vi "Global Log To String(Periodic Check).vi"(0 "Cross CSM Data":T3, 1 "Reset?":bool, 2 "Remove Immediately? (F)":bool, 3 "Time Format String":string="%<%H:%M:%S%3u>T", 9 "Settings":T2={"threashold(#/s)"=1.9, "Check Peroid(s)"=1.0}, 12 "Level (Normal)":T1) -> (4 "String":string, 10 "Periodic Info":string[](array[string]))   [LabVIEW 2017, in "Communicable State Machine.lvlib"]
uses:
  Communicable State Machine.lvlib
  _Support/Typedef/_CSM_GlobalLog_MSG.ctl
  _Support/Typedef/_CSM_Response Source Message.ctl
  _Support/Typedef/_CSM_GlobalLog_MSG_TYPE.ctl
  Periodic String Filter Setting.ctl
  _support/Periodic String Filter Level.ctl
  Periodic String Filter State.ctl
  _Shared/CSM Shared.lvlib
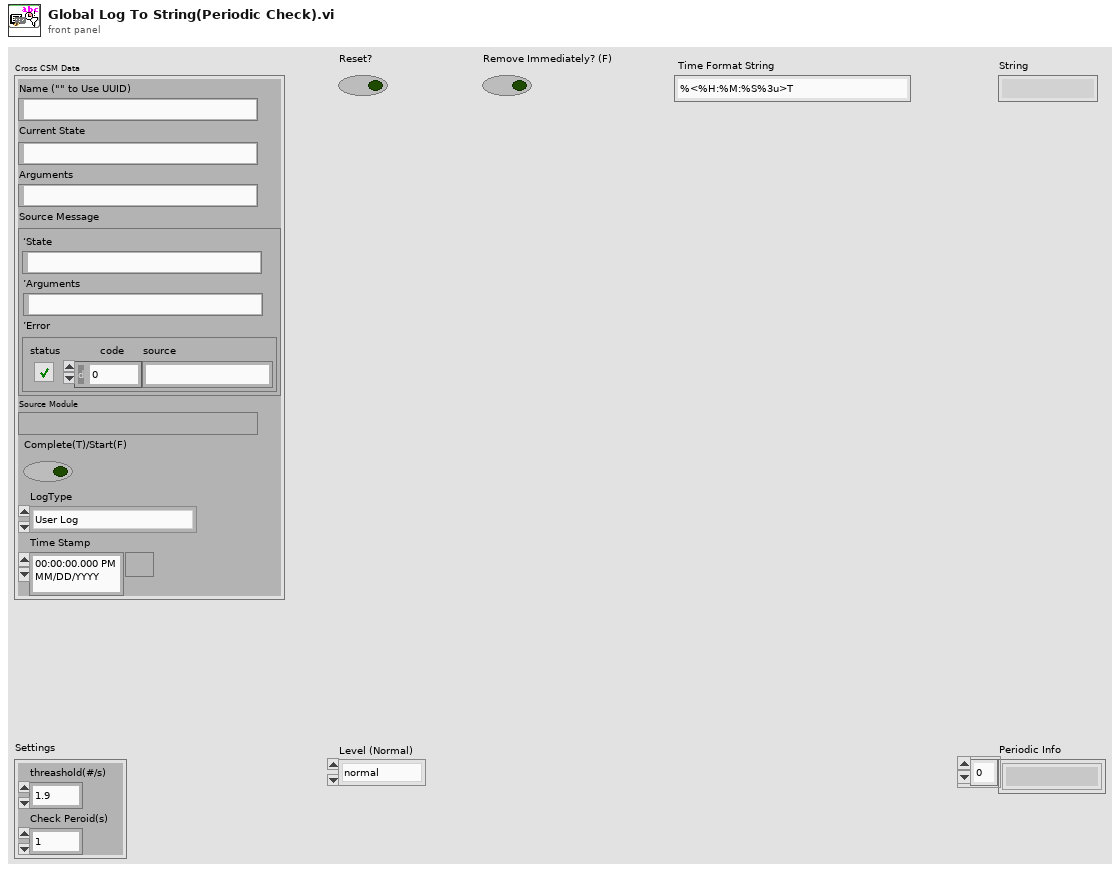
[diagram p1: front panel]
types:
  T1 = typedef "Communicable State Machine.lvlib/Periodic String Filter Level.ctl" = enum16{"normal", "L1", "L2", "L3", "L4"}
  T2 = typedef "Communicable State Machine.lvlib/Periodic String Filter Setting.ctl" = cluster{"threashold(#/s)":dbl, "Check Peroid(s)":dbl}
  T3 = typedef "Communicable State Machine.lvlib/_CSM_GlobalLog_MSG.ctl" = cluster{"Name (\"\" to Use UUID)":string, "Current State":string, "Arguments":string, "Source Message":T4, "Source Module":string, "Complete(T)/Start(F)":bool, "LogType":T5, "Time Stamp":timestamp}
  T4 = typedef "Communicable State Machine.lvlib/_CSM_Response Source Message.ctl" = cluster{"‘State":string, "’Arguments":string, "’Error":errorcluster}
  T5 = typedef "Communicable State Machine.lvlib/_CSM_GlobalLog_MSG_TYPE.ctl" = enum16{"User Log", "State Change", "Status", "Interrupt", "Register", "Unregister", "Error Log", "Module Created", "Module Destroyed", "Async Message", "No-Rep Async Message", "Sync Message", "AsyncMsg Complete", "SyncMsg Complete"}
  T6 = typedef "Communicable State Machine.lvlib/Periodic String Filter State.ctl" = enum16{"Normal", "Remove All Filters"}
  T7 = typedef "Communicable State Machine.lvlib/Periodic String Filter Data.ctl" = cluster{"Keys":string[], "Count":i64[], "LastCheckT":timestamp[], "LastCheckN":i64[], "Filtered":cluster{"Keys":string[], "StartingCount":i64[], "entry":T8[]}}
  T8 = typedef "Communicable State Machine.lvlib/Periodic String Filter Info.ctl" = cluster{"String":string, "Count":i64, "since":timestamp, "param":string, "speed":dbl}
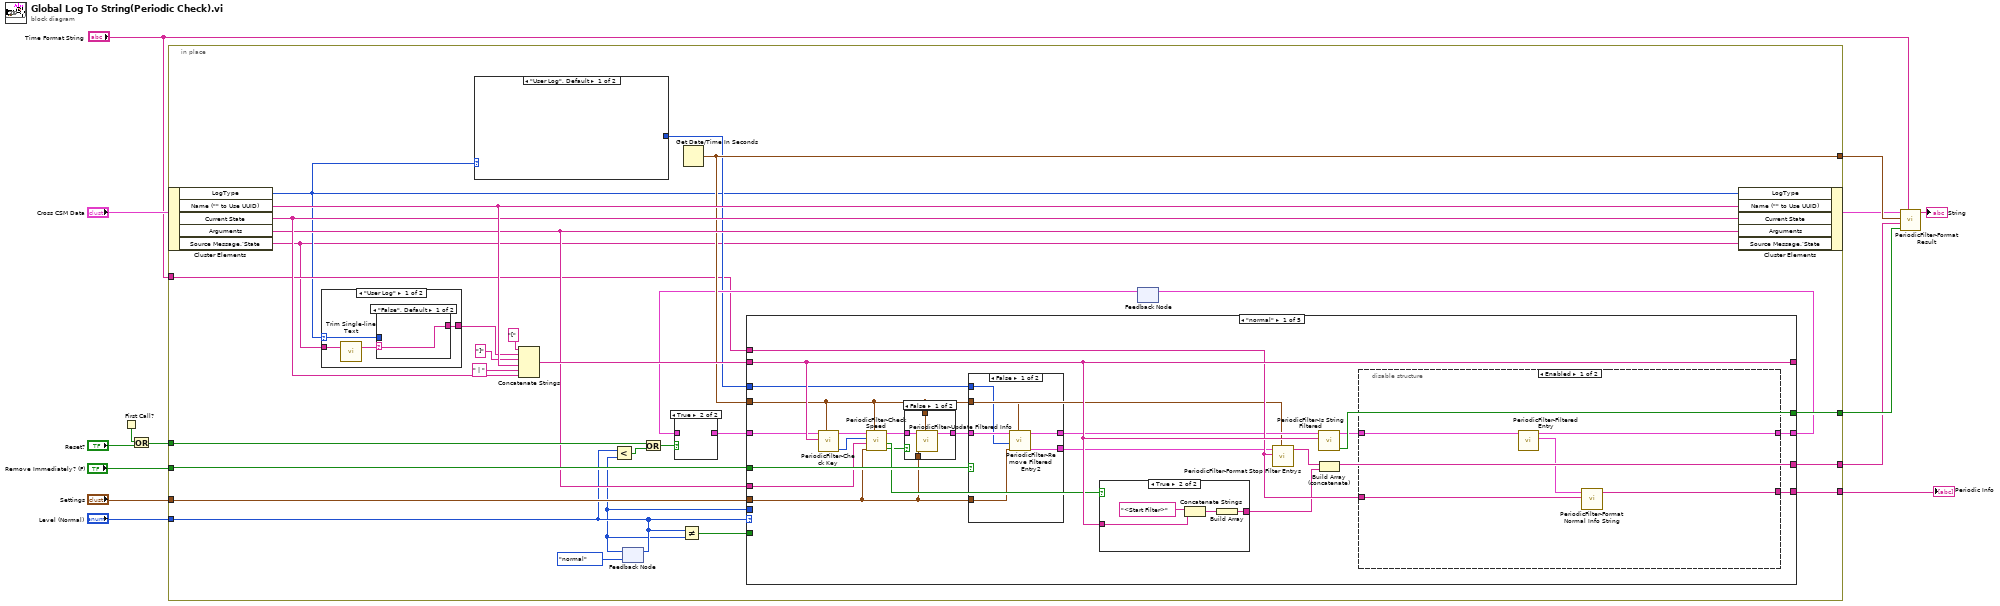
[diagram p0: block diagram]
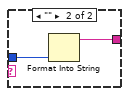
[diagram p2: hidden frame]
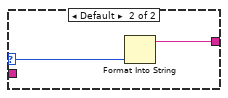
[diagram p3: hidden frame]
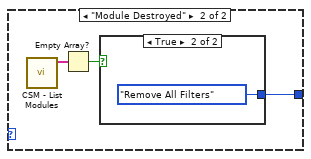
[diagram p4: hidden frame]
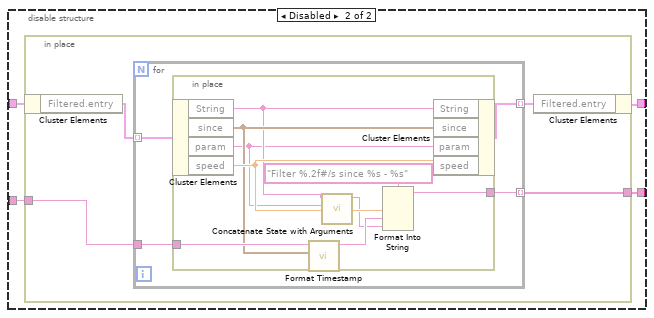
[diagram p7: hidden frame]
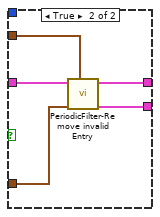
[diagram p8: hidden frame]
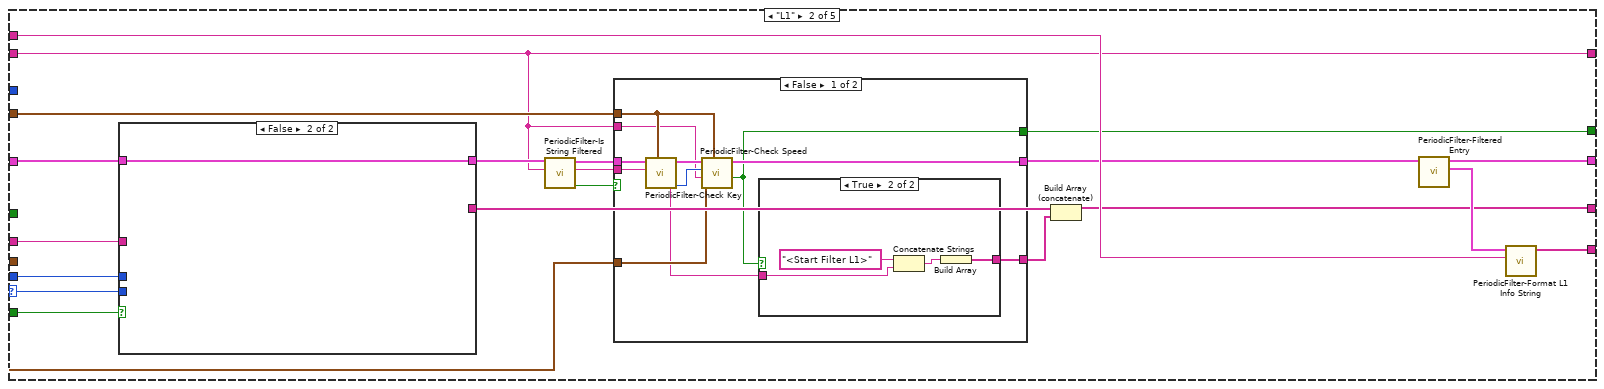
[diagram p10: hidden frame]
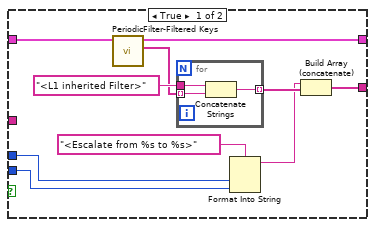
[diagram p13: hidden frame]
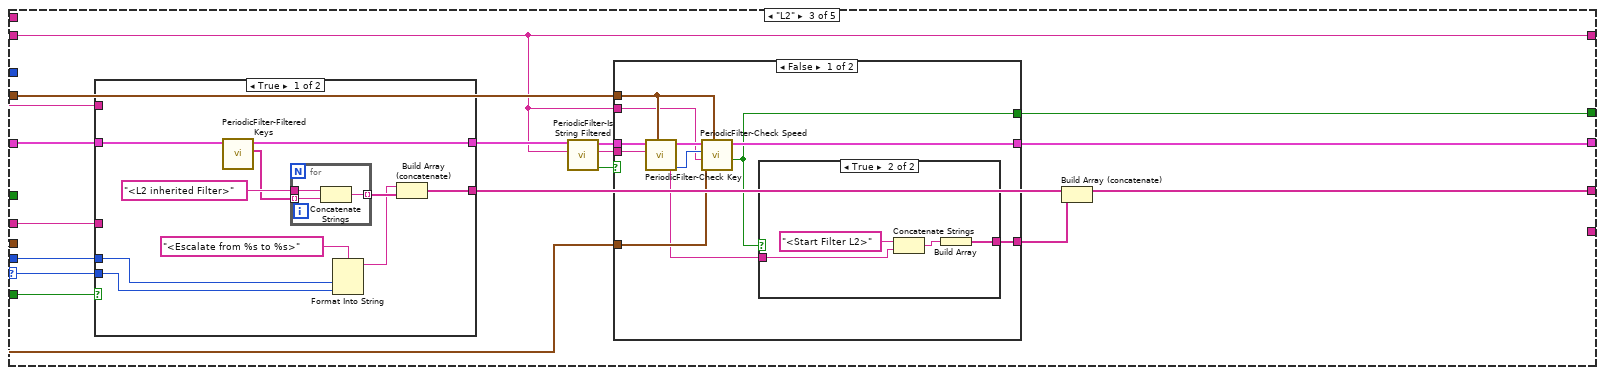
[diagram p14: hidden frame]
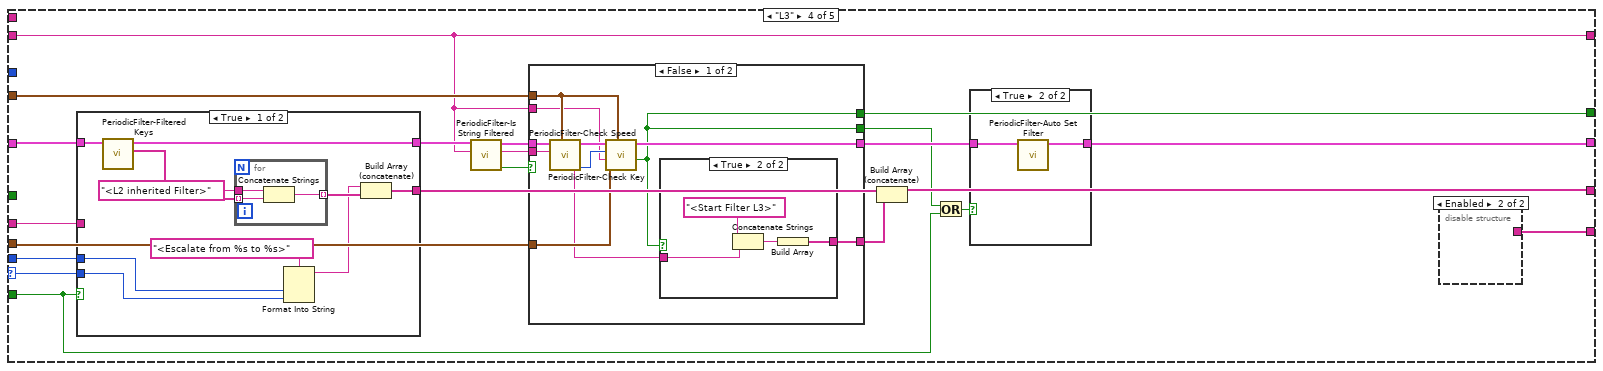
[diagram p18: hidden frame]
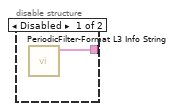
[diagram p19: hidden frame]
diagram:
  n1 = First Call?() -> (First Call?: T/F=w5:bool)
  n2 = Or(x=w5, y="Reset?") -> (x .or. y?=w6:bool)
  n3 = in-place "In Place Element Structure" {
    in-place-border: w6 -> [w39]
    in-place-border: [w37] -> w10
    in-place-border: "Remove Immediately? (F)" -> [w34]
    in-place-border: "Settings" -> [w33]
    in-place-border: "Level (Normal)" -> [w19]
    in-place-border: [w31] -> w9
    in-place-border: [w22] -> w1
    in-place-border: [w21] -> w4
    in-place-border: "Time Format String" -> [w20]
    n4 = in-place-cluster #1("Cross CSM Data") -> ("LogType"=w17:T5, "Name (\"\" to Use UUID)"=w42:string, "Current State"=w41:string, "Arguments"=w32:string, "Source Message.‘State"=w15:string)
    n5 = case shown="\"User Log\"" w17 {
      selector: w17 -> [w45 w50]
      tunnel: [w46 w51] -> w16
      tunnel: w15 -> [w44 _]
      frame "User Log" {
        n6 = call "Trim Single-line Text.vi"("single-line text"=w44) -> ("trimed text"=w43:string)  [unwired: 2 in]
        n7 = case shown="\"False\", Default" w43 {
          selector: w43 -> [w47 _]
          tunnel: [w47 w49] -> w46
          tunnel: w45 -> [_ w48]
          frame "False", Default {
          }
          frame "" {
            n8 = Format Into String(w48) -> (resulting string=w49:string)  [unwired: 3 in, 1 out]
          }
        }
      }
      frame Default {
        n9 = Format Into String(w50) -> (resulting string=w51:string)  [unwired: 3 in, 1 out]
      }
    }
    n10 = case shown="\"User Log\", Default" w17 {
      tunnel: [_ w52] -> w23
      frame "User Log", Default {
      }
      frame "Module Destroyed" {
        n11 = call "CSM - List Modules.vi"() -> ("Module Names"=w54:string[])  [unwired: 10 in, 1 out]
        n12 = Empty Array?(array=w54) -> (empty?=w53:bool)
        n13 = case shown="True" w53 {
          tunnel: [_ Periodic_String_Filter_State."Remove All Filters" ("State")] -> w52
          frame False {
          }
          frame True {
          }
        }
      }
    }
    n14 = Concatenate Strings("[" ("string"), w16, "]" ("string"), w42, " | " ("string"), w41) -> (w38:string)
    n15 = feedback #2(Periodic_String_Filter_Level."normal" ("Level(Normal)")) -> (w18:T1)
    n16 = Less?(x=w19, y=w18) -> (x < y?=w29:bool)
    n17 = feedback-in #2(w19) -> ()
    n18 = Or(x=w39, y=w29) -> (x .or. y?=w24:bool)
    n19 = Not Equal?(x=w19, y=w18) -> (x != y?=w28:bool)
    n20 = Get Date/Time In Seconds() -> (seconds since 1Jan1904=w31:timestamp)
    n21 = feedback #3() -> (w27:T7)  [unwired: 1 in]
    n22 = case shown="True" w24 {
      tunnel: [w288 _] -> w26
      tunnel: w27 -> [w288 _]
      frame False {
      }
      frame True {
      }
    }
    n23 = case shown="\"normal\"" w19 {
      selector: w19 -> [_ w125 w176 w223 _]
      tunnel: w38 -> [w78 w127 w178 w230 w283]
      tunnel: [w78 w127 w178 w230 w283] -> _
      tunnel: w33 -> [w58 w131 w182 w233 _]
      tunnel: w31 -> [w56 w132 w183 w234 _]
      tunnel: [w76 w138 w185 w229 w279] -> w25
      tunnel: w26 -> [w75 w145 w192 w243 w281]
      tunnel: [w74 w130 w181 w227 TRUE ("new filtered Item")] -> w37
      tunnel: w34 -> [w77 _ _ _ _]
      tunnel: w28 -> [_ w144 w191 w228 w280]
      tunnel: w32 -> [w73 w143 w190 w242 _]
      tunnel: w23 -> [w72 _ _ _ _]
      tunnel: [w71 w142 _ w241 _] -> w22
      tunnel: [w70 w129 w180 w232 w278] -> w21
      tunnel: w20 -> [w69 w141 _ _ _]
      tunnel: w18 -> [_ w126 w177 w224 _]
      frame "normal" {
        n24 = call "PeriodicFilter-Check Key.vi"("Seconds Since 1Jan1904 2"=w56, "Key"=w78, "Data In"=w75) -> ("Index"=w68:i32, "Data Out"=w67:T7)  [unwired: 7 in]
        n25 = call "PeriodicFilter-Check Speed.vi"("Seconds Since 1Jan1904"=w56, "Settings"=w58, "Parameter"=w73, "Index"=w68, "Data In"=w67) -> ("Over Threshold?"=w57:bool, "New Filtered Item"=w64:bool, "Data Out"=w66:T7)  [unwired: 4 in]
        n26 = case shown="False" w57 {
          tunnel: w66 -> [w82 w83]
          tunnel: [w81 w83] -> w65
          tunnel: w56 -> [w80 _]
          tunnel: w58 -> [w79 _]
          frame False {
            n27 = call "PeriodicFilter-Update Filtered Info.vi"("Seconds Since 1Jan1904"=w80, "Settings"=w79, "Data In"=w82) -> ("Data Out"=w81:T7)  [unwired: 8 in]
          }
          frame True {
          }
        }
        n28 = case shown="False" w77 {
          tunnel: w65 -> [w115 w120]
          tunnel: w56 -> [w114 w119]
          tunnel: [w113 w118] -> w63
          tunnel: [w112 w117] -> w62
          tunnel: w58 -> [w110 w116]
          tunnel: w72 -> [w111 _]
          frame False {
            n29 = call "PeriodicFilter-Remove Filtered Entry2.vi"("Seconds Since 1Jan1904 2"=w114, "Settings"=w110, "State"=w111, "Data In"=w115) -> ("Removed Info"=w112:T8[], "Data Out"=w113:T7)  [unwired: 6 in]
          }
          frame True {
            n30 = call "PeriodicFilter-Remove invalid Entry.vi"("Seconds Since 1Jan1904 2"=w119, "Settings"=w116, "Data In"=w120) -> ("Removed Info"=w117:T8[], "Data Out"=w118:T7)  [unwired: 7 in]
          }
        }
        n31 = case shown="True" w64 {
          tunnel: [_ w124] -> w60
          tunnel: w78 -> [_ w122]
          frame False {
          }
          frame True {
            n32 = Concatenate Strings("<Start Filter>" ("Current State"), w122) -> (w121:string)
            n33 = Build Array(w121) -> (w124:string[])
          }
        }
        n34 = call "PeriodicFilter-Format Stop Filter Entrys.vi"("Seconds Since 1Jan1904 2"=w56, "Time Format String"=w69, "Removed Info"=w62) -> ("Array"=w59:string[])  [unwired: 8 in]
        n35 = call "PeriodicFilter-Is String Filtered.vi"("Input String"=w78, "Data In"=w63) -> ("Filtered"=w74:bool, "Data Out"=w61:T7)  [unwired: 7 in, 1 out]
        n36 = Build Array (concatenate)(w59, w60) -> (w70:string[])
        n37 = disable-structure shown="Enabled" {
          disable-tunnel: [w88 w91] -> w76
          disable-tunnel: [w87 w89] -> w71
          disable-tunnel: w69 -> [w86 w90]
          disable-tunnel: w61 -> [w85 w92]
          frame Enabled {
            n38 = call "PeriodicFilter-Filtered Entry.vi"("Data In"=w85) -> ("Entry"=w84:T8[], "Data Out"=w88:T7)  [unwired: 9 in]
            n39 = call "PeriodicFilter-Format Normal Info String.vi"("Time Format String"=w86, "Removed Info"=w84) -> ("Array"=w87:string[])  [unwired: 9 in]
          }
          frame Disabled {
            n40 = in-place {
              in-place-border: w90 -> [w95]
              in-place-border: [w94] -> w89
              n41 = in-place-cluster #4(w92) -> ("Filtered.entry"=w96:T8[])
              n42 = for {
                tunnel: w96 -> [w98] mode=indexing
                tunnel: [w100] -> w94 mode=indexing
                tunnel: w95 -> [w99]
                tunnel: [w97] -> w93 mode=indexing
                n43 = in-place {
                  in-place-border: [w109] -> w100
                  in-place-border: w99 -> [w106]
                  n44 = in-place-cluster #5(w98) -> ("String"=w103:string, "since"=w104:timestamp, "param"=w101:string, "speed"=w105:dbl)
                  n45 = call "Format Timestamp.vi"("Timestamp"=w104, "Format String"=w106) -> ("String"=w107:string)  [unwired: 9 in]
                  n46 = call "Concatenate State with Arguments.vi"("Arguments"=w101, "State"=w103) -> ("State With Arguements"=w102:string)  [unwired: 9 in]
                  n47 = Format Into String(format string="Filter %.2f#/s since %s - %s", w105, w107, w102) -> (resulting string=w109:string)  [unwired: 2 in, 1 out]
                  n48 = in-place-cluster #5("String"=w103, "since"=w104, "param"=w101, "speed"=w105) -> (w97:T8)
                }
              }
              n49 = in-place-cluster #4("Filtered.entry"=w93) -> (w91:T7)
            }
          }
        }
      }
      frame "L1" {
        n50 = case shown="False" w144 {
          tunnel: w145 -> [w171 w175]
          tunnel: [w166 w175] -> w133
          tunnel: [w167 _] -> w140
          tunnel: w143 -> [_ _]
          tunnel: w126 -> [w164 _]
          tunnel: w125 -> [w163 _]
          frame True {
            n51 = call "PeriodicFilter-Filtered Keys.vi"("Data In"=w171) -> ("Filtered Keys"=w169:string[], "Data Out"=w166:T7)  [unwired: 9 in]
            n52 = for {
              tunnel: w169 -> [w174] mode=indexing
              tunnel: [w173] -> w168 mode=indexing
              tunnel: "<L1 inherited Filter>" ("Current State") -> [w172]
              n53 = Concatenate Strings(w172, w174) -> (w173:string)
            }
            n54 = Format Into String(format string="<Escalate from %s to %s>" ("Current State"), w164, w163) -> (resulting string=w162:string)  [unwired: 2 in, 1 out]
            n55 = Build Array (concatenate)(w162, w168) -> (w167:string[])
          }
          frame False {
          }
        }
        n56 = call "PeriodicFilter-Is String Filtered.vi"("Input String"=w127, "Data In"=w133) -> ("Filtered"=w135:bool, "Input String (Dup)"=w137:string, "Data Out"=w136:T7)  [unwired: 7 in]
        n57 = case shown="False" w135 {
          selector: w135 -> [_ w160]
          tunnel: w136 -> [w153 w161]
          tunnel: [w152 w161] -> w134
          tunnel: w132 -> [w151 _]
          tunnel: w137 -> [w146 _]
          tunnel: [w150 _] -> w128
          tunnel: [w149 w160] -> w130
          tunnel: w131 -> [w148 _]
          tunnel: w127 -> [w147 _]
          frame False {
            n58 = call "PeriodicFilter-Check Key.vi"("Seconds Since 1Jan1904 2"=w151, "Key"=w146, "Data In"=w153) -> ("Index"=w154:i32, "Data Out"=w155:T7)  [unwired: 7 in]
            n59 = call "PeriodicFilter-Check Speed.vi"("Seconds Since 1Jan1904"=w151, "Settings"=w148, "Parameter"=w147, "Index"=w154, "Data In"=w155) -> ("New Filtered Item"=w149:bool, "Data Out"=w152:T7)  [unwired: 4 in, 1 out]
            n60 = case shown="True" w149 {
              tunnel: [_ w156] -> w150
              tunnel: w146 -> [_ w159]
              frame False {
              }
              frame True {
                n61 = Concatenate Strings("<Start Filter L1>" ("Current State"), w159) -> (w157:string)
                n62 = Build Array(w157) -> (w156:string[])
              }
            }
          }
          frame True {
          }
        }
        n63 = Build Array (concatenate)(w140, w128) -> (w129:string[])
        n64 = call "PeriodicFilter-Filtered Entry.vi"("Data In"=w134) -> ("Entry"=w139:T8[], "Data Out"=w138:T7)  [unwired: 9 in]
        n65 = call "PeriodicFilter-Format L1 Info String.vi"("Time Format String"=w141, "Entry"=w139) -> ("Array"=w142:string[])  [unwired: 9 in]
      }
      frame "L2" {
        n66 = case shown="True" w191 {
          tunnel: w192 -> [w218 w222]
          tunnel: [w213 w222] -> w184
          tunnel: w178 -> [_ _]
          tunnel: [w214 _] -> w189
          tunnel: w190 -> [_ _]
          tunnel: w177 -> [w211 _]
          tunnel: w176 -> [w210 _]
          frame True {
            n67 = call "PeriodicFilter-Filtered Keys.vi"("Data In"=w218) -> ("Filtered Keys"=w216:string[], "Data Out"=w213:T7)  [unwired: 9 in]
            n68 = for {
              tunnel: w216 -> [w221] mode=indexing
              tunnel: [w220] -> w215 mode=indexing
              tunnel: "<L2 inherited Filter>" ("Current State") -> [w219]
              n69 = Concatenate Strings(w219, w221) -> (w220:string)
            }
            n70 = Format Into String(format string="<Escalate from %s to %s>" ("Current State"), w211, w210) -> (resulting string=w209:string)  [unwired: 2 in, 1 out]
            n71 = Build Array (concatenate)(w209, w215) -> (w214:string[])
          }
          frame False {
          }
        }
        n72 = call "PeriodicFilter-Is String Filtered.vi"("Input String"=w178, "Data In"=w184) -> ("Filtered"=w186:bool, "Input String (Dup)"=w188:string, "Data Out"=w187:T7)  [unwired: 7 in]
        n73 = case shown="False" w186 {
          selector: w186 -> [_ w207]
          tunnel: w187 -> [w200 w208]
          tunnel: [w199 w208] -> w185
          tunnel: w183 -> [w198 _]
          tunnel: w188 -> [w193 _]
          tunnel: [w197 _] -> w179
          tunnel: [w196 w207] -> w181
          tunnel: w182 -> [w195 _]
          tunnel: w178 -> [w194 _]
          frame False {
            n74 = call "PeriodicFilter-Check Key.vi"("Seconds Since 1Jan1904 2"=w198, "Key"=w193, "Data In"=w200) -> ("Index"=w201:i32, "Data Out"=w202:T7)  [unwired: 7 in]
            n75 = call "PeriodicFilter-Check Speed.vi"("Seconds Since 1Jan1904"=w198, "Settings"=w195, "Parameter"=w194, "Index"=w201, "Data In"=w202) -> ("New Filtered Item"=w196:bool, "Data Out"=w199:T7)  [unwired: 4 in, 1 out]
            n76 = case shown="True" w196 {
              tunnel: [_ w203] -> w197
              tunnel: w193 -> [_ w206]
              frame False {
              }
              frame True {
                n77 = Concatenate Strings("<Start Filter L2>" ("Current State"), w206) -> (w204:string)
                n78 = Build Array(w204) -> (w203:string[])
              }
            }
          }
          frame True {
          }
        }
        n79 = Build Array (concatenate)(w189, w179) -> (w180:string[])
      }
      frame "L3" {
        n80 = case shown="True" w228 {
          tunnel: w243 -> [w270 w277]
          tunnel: [w269 w277] -> w235
          tunnel: [w273 _] -> w240
          tunnel: w242 -> [_ _]
          tunnel: w224 -> [w266 _]
          tunnel: w223 -> [w265 _]
          frame True {
            n81 = call "PeriodicFilter-Filtered Keys.vi"("Data In"=w270) -> ("Filtered Keys"=w272:string[], "Data Out"=w269:T7)  [unwired: 9 in]
            n82 = for {
              tunnel: w272 -> [w276] mode=indexing
              tunnel: [w275] -> w268 mode=indexing
              tunnel: "<L2 inherited Filter>" ("Current State") -> [w274]
              n83 = Concatenate Strings(w274, w276) -> (w275:string)
            }
            n84 = Format Into String(format string="<Escalate from %s to %s>" ("Current State"), w266, w265) -> (resulting string=w264:string)  [unwired: 2 in, 1 out]
            n85 = Build Array (concatenate)(w264, w268) -> (w273:string[])
          }
          frame False {
          }
        }
        n86 = call "PeriodicFilter-Is String Filtered.vi"("Input String"=w230, "Data In"=w235) -> ("Filtered"=w237:bool, "Input String (Dup)"=w239:string, "Data Out"=w238:T7)  [unwired: 7 in]
        n87 = case shown="False" w237 {
          selector: w237 -> [_ w262]
          tunnel: w238 -> [w255 w263]
          tunnel: [w254 w263] -> w236
          tunnel: w234 -> [w253 _]
          tunnel: w239 -> [w249 _]
          tunnel: [w252 _] -> w231
          tunnel: [w248 w262] -> w227
          tunnel: w233 -> [w251 _]
          tunnel: w230 -> [w250 _]
          tunnel: [w248 _] -> w225
          frame False {
            n88 = call "PeriodicFilter-Check Key.vi"("Seconds Since 1Jan1904 2"=w253, "Key"=w249, "Data In"=w255) -> ("Index"=w256:i32, "Data Out"=w257:T7)  [unwired: 7 in]
            n89 = call "PeriodicFilter-Check Speed.vi"("Seconds Since 1Jan1904"=w253, "Settings"=w251, "Parameter"=w250, "Index"=w256, "Data In"=w257) -> ("New Filtered Item"=w248:bool, "Data Out"=w254:T7)  [unwired: 4 in, 1 out]
            n90 = case shown="True" w248 {
              tunnel: [_ w258] -> w252
              tunnel: w249 -> [_ w261]
              frame False {
              }
              frame True {
                n91 = Concatenate Strings("<Start Filter L3>" ("Current State"), w261) -> (w259:string)
                n92 = Build Array(w259) -> (w258:string[])
              }
            }
          }
          frame True {
          }
        }
        n93 = Build Array (concatenate)(w240, w231) -> (w232:string[])
        n94 = Or(x=w225, y=w228) -> (x .or. y?=w226:bool)
        n95 = case shown="True" w226 {
          tunnel: w236 -> [w245 w247]
          tunnel: [w245 w246] -> w229
          frame False {
          }
          frame True {
            n96 = call "PeriodicFilter-Auto Set Filter.vi"("Data In"=w247) -> ("Data Out"=w246:T7)  [unwired: 10 in]
          }
        }
        n97 = disable-structure shown="Enabled" {
          disable-tunnel: [w244 _] -> w241
          frame Disabled {
            n98 = call "PeriodicFilter-Format L3 Info String.vi"() -> ("Array"=w244:string[])  [unwired: 11 in]
          }
          frame Enabled {
          }
        }
      }
      frame Default {
        n99 = case shown="True" w280 {
          tunnel: w281 -> [w284 w287]
          tunnel: [w284 w287] -> w279
          tunnel: [w285 _] -> w278
          frame True {
            n100 = Build Array("<Escalate from Top Level, All messages are filtered.>" ("Current State")) -> (w285:string[])
          }
          frame False {
          }
        }
      }
    }
    n101 = feedback-in #3(w25) -> ()
    n102 = in-place-cluster #1("LogType"=w17, "Name (\"\" to Use UUID)"=w42, "Current State"=w41, "Arguments"=w32, "Source Message.‘State"=w15) -> (w8:T3)
  }
  "Periodic Info" <- w1
  n103 = call "PeriodicFilter-Format Result.vi"("Time Format String"="Time Format String", "Filtered"=w10, "Additional Info"=w4, "Current Time"=w9, "Cross CSM Data In"=w8) -> ("States"=→"String":string)  [unwired: 6 in]
